vi "from string 3.0.vi"(8 "error in":errorcluster, 10 "data in":string, 11 "Shared Memory configuration in":refnum<class "Shared Memory configuration.lvclass">) -> (0 "error out":errorcluster, 2 "remaining data":string, 3 "Shared Memory configuration out":refnum<class "Shared Memory configuration.lvclass">)   [LabVIEW 2014, in "Shared Memory configuration.lvclass"]
uses:
  Shared Memory configuration.lvclass
  editor node/sync/sync item.ctl
  editor node/sync/sync mechanism.ctl
  Shared Memory configuration.lvclass/Shared Memory configuration.ctl
  <vilib>/NI/Configuration Framework/serializable configuration/NISE_CEF_serializable configuration.lvclass
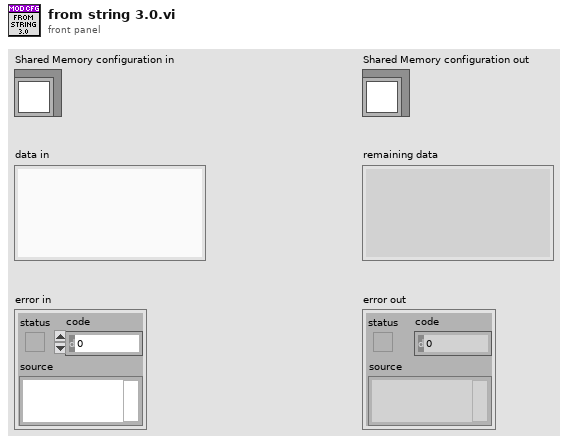
[diagram p1: front panel]
types:
  T1 = typedef "Shared Memory configuration.lvclass/sync item.ctl" = cluster{"mechanism":T2, "name":string}
  T2 = typedef "Shared Memory configuration.lvclass/sync mechanism.ctl" = enum16{"Semaphore"}
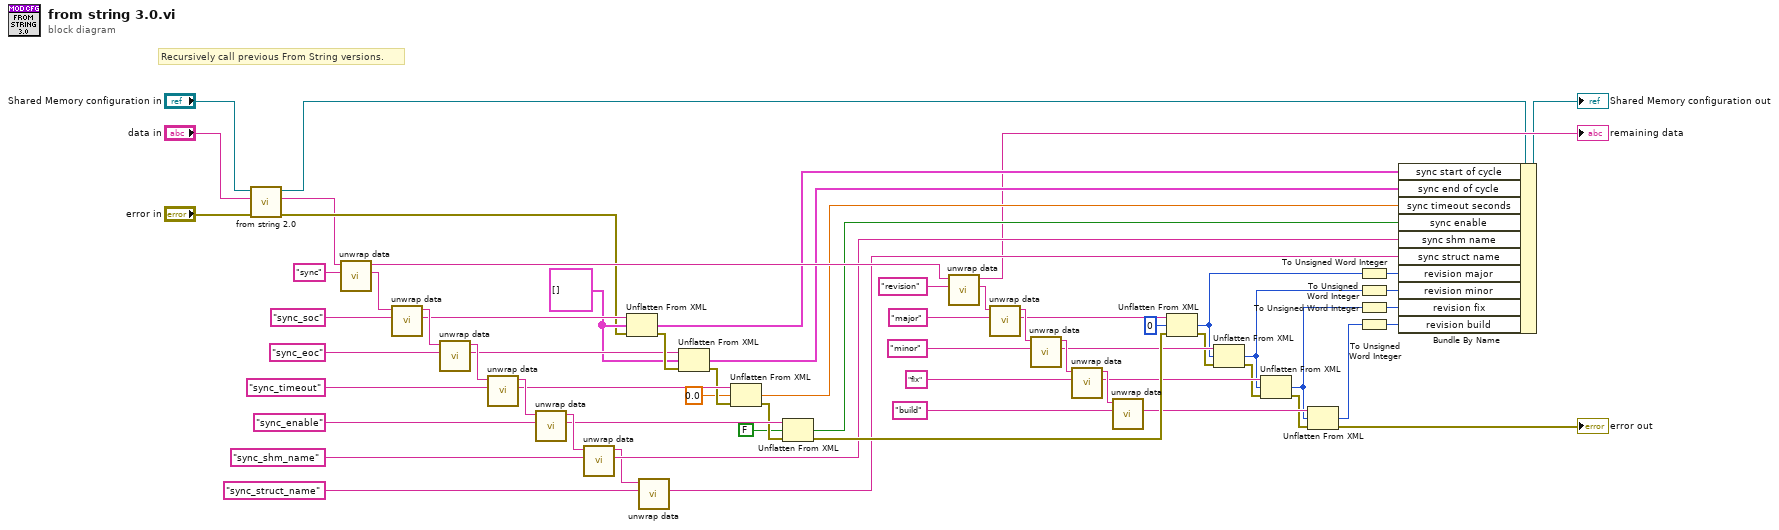
[diagram p0: block diagram]
diagram:
  w46 = T1[] [] ("sync start of cycle")
  # "Recursively call previous From String versions."
  n1 = call "from string 2.0.vi"("error in"="error in", "data in"="data in", "Shared Memory configuration in"="Shared Memory configuration in") -> ("error out"=w13:errorcluster, "remaining data"=w12:string, "Shared Memory configuration out"=w10:refnum<class "Shared Memory configuration.lvclass">)  [unwired: 6 in]
  n2 = call <vilib>:"unwrap data.vi"("identifier"="sync", "data to unwrap"=w12) -> ("unwrapped data"=w52:string, "remaining string"=w58:string)  [unwired: 8 in]
  n3 = call <vilib>:"unwrap data.vi"("identifier"="sync_soc", "data to unwrap"=w52) -> ("unwrapped data"=w48:string, "remaining string"=w51:string)  [unwired: 8 in]
  n4 = call <vilib>:"unwrap data.vi"("identifier"="sync_eoc", "data to unwrap"=w51) -> ("unwrapped data"=w47:string, "remaining string"=w50:string)  [unwired: 8 in]
  n5 = call <vilib>:"unwrap data.vi"("identifier"="sync_timeout", "data to unwrap"=w50) -> ("unwrapped data"=w45:string, "remaining string"=w49:string)  [unwired: 8 in]
  n6 = call <vilib>:"unwrap data.vi"("identifier"="sync_enable", "data to unwrap"=w49) -> ("unwrapped data"=w43:string, "remaining string"=w44:string)  [unwired: 8 in]
  n7 = call <vilib>:"unwrap data.vi"("identifier"="sync_shm_name", "data to unwrap"=w44) -> ("unwrapped data"=w34:string, "remaining string"=w16:string)  [unwired: 8 in]
  n8 = Unflatten From XML(xml string=w48, type=w46, error in (no error)=w13) -> (value=w38:T1[], error out=w61:errorcluster)
  n9 = call <vilib>:"unwrap data.vi"("identifier"="sync_struct_name", "data to unwrap"=w16) -> ("unwrapped data"=w15:string)  [unwired: 8 in, 1 out]
  n10 = Unflatten From XML(xml string=w47, type=w46, error in (no error)=w61) -> (value=w37:T1[], error out=w42:errorcluster)
  n11 = Unflatten From XML(xml string=w45, type=0.0, error in (no error)=w42) -> (value=w36:dbl, error out=w41:errorcluster)
  n12 = Unflatten From XML(xml string=w43, type=FALSE, error in (no error)=w41) -> (value=w35:bool, error out=w62:errorcluster)
  n13 = call <vilib>:"unwrap data.vi"("identifier"="revision", "data to unwrap"=w58) -> ("unwrapped data"=w18:string, "remaining string"=→"remaining data":string)  [unwired: 8 in]
  n14 = call <vilib>:"unwrap data.vi"("identifier"="major", "data to unwrap"=w18) -> ("unwrapped data"=w27:string, "remaining string"=w33:string)  [unwired: 8 in]
  n15 = call <vilib>:"unwrap data.vi"("identifier"="minor", "data to unwrap"=w33) -> ("unwrapped data"=w28:string, "remaining string"=w32:string)  [unwired: 8 in]
  n16 = call <vilib>:"unwrap data.vi"("identifier"="fix", "data to unwrap"=w32) -> ("unwrapped data"=w29:string, "remaining string"=w31:string)  [unwired: 8 in]
  n17 = call <vilib>:"unwrap data.vi"("identifier"="build", "data to unwrap"=w31) -> ("unwrapped data"=w30:string)  [unwired: 8 in, 1 out]
  n18 = Unflatten From XML(xml string=w27, type=u8 0, error in (no error)=w62) -> (value=w1:u8, error out=w22:errorcluster)
  n19 = Unflatten From XML(xml string=w28, type=w1, error in (no error)=w22) -> (value=w2:u8, error out=w21:errorcluster)
  n20 = Unflatten From XML(xml string=w29, type=w2, error in (no error)=w21) -> (value=w3:u8, error out=w20:errorcluster)
  n21 = Unflatten From XML(xml string=w30, type=w3, error in (no error)=w20) -> (value=w8:u8, error out=→"error out":errorcluster)
  n22 = To Unsigned Word Integer(number=w1) -> (unsigned 16bit integer=w4:u16)
  n23 = To Unsigned Word Integer(number=w2) -> (unsigned 16bit integer=w5:u16)
  n24 = To Unsigned Word Integer(number=w3) -> (unsigned 16bit integer=w6:u16)
  n25 = To Unsigned Word Integer(number=w8) -> (unsigned 16bit integer=w7:u16)
  n26 = Bundle By Name(cluster=w10, "sync start of cycle"=w38, "sync end of cycle"=w37, "sync timeout seconds"=w36, "sync enable"=w35, "sync shm name"=w34, "sync struct name"=w15, "revision major"=w4, "revision minor"=w5, "revision fix"=w6, "revision build"=w7) -> (→"Shared Memory configuration out":refnum<class "Shared Memory configuration.lvclass">)
